vi "Resolve URL.vi"(10 "Path":string, 11 "REST Client in":refnum<class "REST Client.lvclass">) -> (2 "Resolved URL":string)   [LabVIEW 2020, in "REST Client.lvlib" / "REST Client.lvclass"]
uses:
  REST Client.lvclass
  REST Client.lvclass/REST Client.ctl
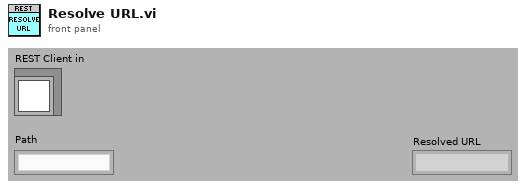
[diagram p1: front panel]
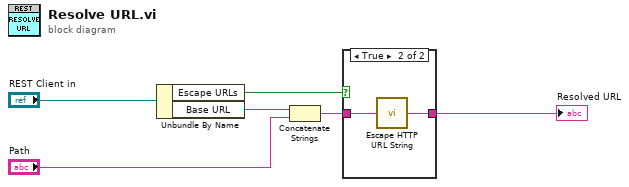
[diagram p0: block diagram]
diagram:
  n1 = Unbundle By Name("REST Client in") -> ("Escape URLs"=w1:bool, "Base URL"=w2:string)
  n2 = Concatenate Strings(w2, "Path") -> (w3:string)
  n3 = case shown="True" w1 {
    tunnel: w3 -> [w7 w9]
    tunnel: [w7 w8] -> w4
    frame False {
    }
    frame True {
      n4 = call "Escape HTTP URL String.vi"("Unescaped HTTP URL string in"=w9) -> ("Escaped HTTP URL string out"=w8:string)
    }
  }
  "Resolved URL" <- w4
